vi "Plot menu activation.vi"(5 "panel mode":T1, 8 "error in (no error)":errorcluster, 9 "Coords":T5, 10 "Refs":T6, 11 "MenuRef":refnum<k9>) -> (0 "error out":errorcluster, 1 "Location":T2, 2 "Discard?":bool, 3 "MenuRef":refnum<k9>)   [LabVIEW 2021, in "RocketPlot.lvlib"]
uses:
  RocketPlot.lvlib
  Classes/RocketPlotHandle/RocketPlotHandle.lvclass
  TypeDefs/Plot UI references.ctl
  <userlib>/bjustice/TipStripOOPanel/Classes/TipPanelHandle/TipPanelHandle.lvclass
  TypeDefs/Plot top row.ctl
  <vilib>/Utility/miscctls.llb/LVPoint32TypeDef.ctl
  TypeDefs/Shortcut Location.ctl
  Plot menu activation submenu type v2.ctl
  TypeDefs/Plot axis.ctl
  Plot scale refnum to LUT name.vi
  TypeDefs/panel mode.ctl
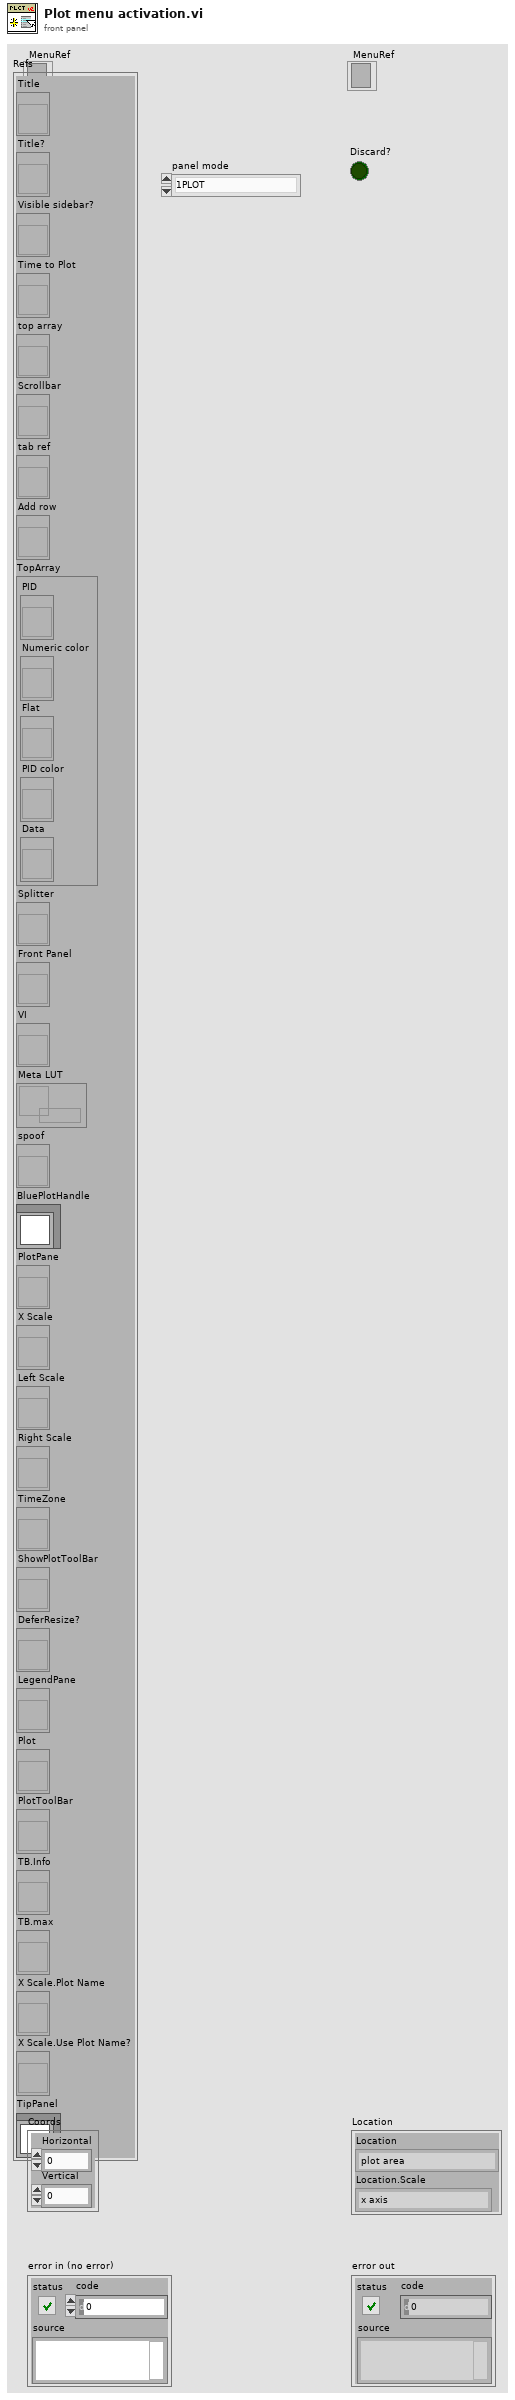
[diagram p1: front panel]
types:
  T1 = typedef "RocketPlot.lvlib/panel mode.ctl" = enum16{"1PLOT", "MPLOT"}
  T2 = typedef "RocketPlot.lvlib/Shortcut Location.ctl" = cluster{"Location":T3, "Location.Scale":T4}
  T3 = typedef "RocketPlot.lvlib/Plot menu activation submenu type v2.ctl" = enum16{"plot area", "plot border", "markers", "scale"}
  T4 = typedef "RocketPlot.lvlib/Plot axis.ctl" = enum16{"x axis", "left axis", "right axis"}
  T5 = typedef "LVPoint32TypeDef.ctl" = cluster{"Horizontal":i32, "Vertical":i32}
  T6 = typedef "RocketPlot.lvlib/Plot UI references.ctl" = cluster{"Title":refnum<vi>, "Title?":refnum<vi>, "Visible sidebar?":refnum<vi>, "Time to Plot":refnum<vi>, "top array":refnum<vi>, "Scrollbar":refnum<vi>, "tab ref":refnum<vi>, "Add row":refnum<vi>, "TopArray":cluster{"PID":refnum<vi>, "Numeric color":refnum<vi>, "Flat":refnum<vi>, "PID color":refnum<vi>, "Data":refnum<vi>}, "Splitter":refnum<vi>, "Front Panel":refnum<vi>, "VI":refnum<vi>, "Meta LUT":refnum<data-value>, "spoof":refnum<vi>, "BluePlotHandle":refnum<class "RocketPlotHandle.lvclass">, "PlotPane":refnum<vi>, "X Scale":refnum<vi>, "Left Scale":refnum<vi>, "Right Scale":refnum<vi>, "TimeZone":refnum<vi>, "ShowPlotToolBar":refnum<vi>, "DeferResize?":refnum<vi>, "LegendPane":refnum<vi>, "Plot":refnum<vi>, "PlotToolBar":refnum<vi>, "TB.Info":refnum<vi>, "TB.max":refnum<vi>, "X Scale.Plot Name":refnum<vi>, "X Scale.Use Plot Name?":refnum<vi>, "TipPanel":refnum<class "TipPanelHandle.lvclass">}
  T7 = typedef "RocketPlot.lvlib/PlatMods.ctl" = cluster{"Shift":bool, "Ctrl":bool, "Alt":bool}
  T8 = typedef "RocketPlot.lvlib/Plot scale meta JSON.ctl" = cluster{"Type":T4, "Grid Colors:Major Color":u32, "Grid Colors:Minor Color":u32, "Style":u8, "Tick Colors:Tick Color":u32, "Tick Colors:Minor Tick Color":u32, "Format String":string, "State":T9, "AxisFocus":refnum<vi>}
  T9 = typedef "RocketPlot.lvlib/Plot scale meta state.ctl" = cluster{"Visible":bool, "Focus":bool, "Multi-Y":bool}
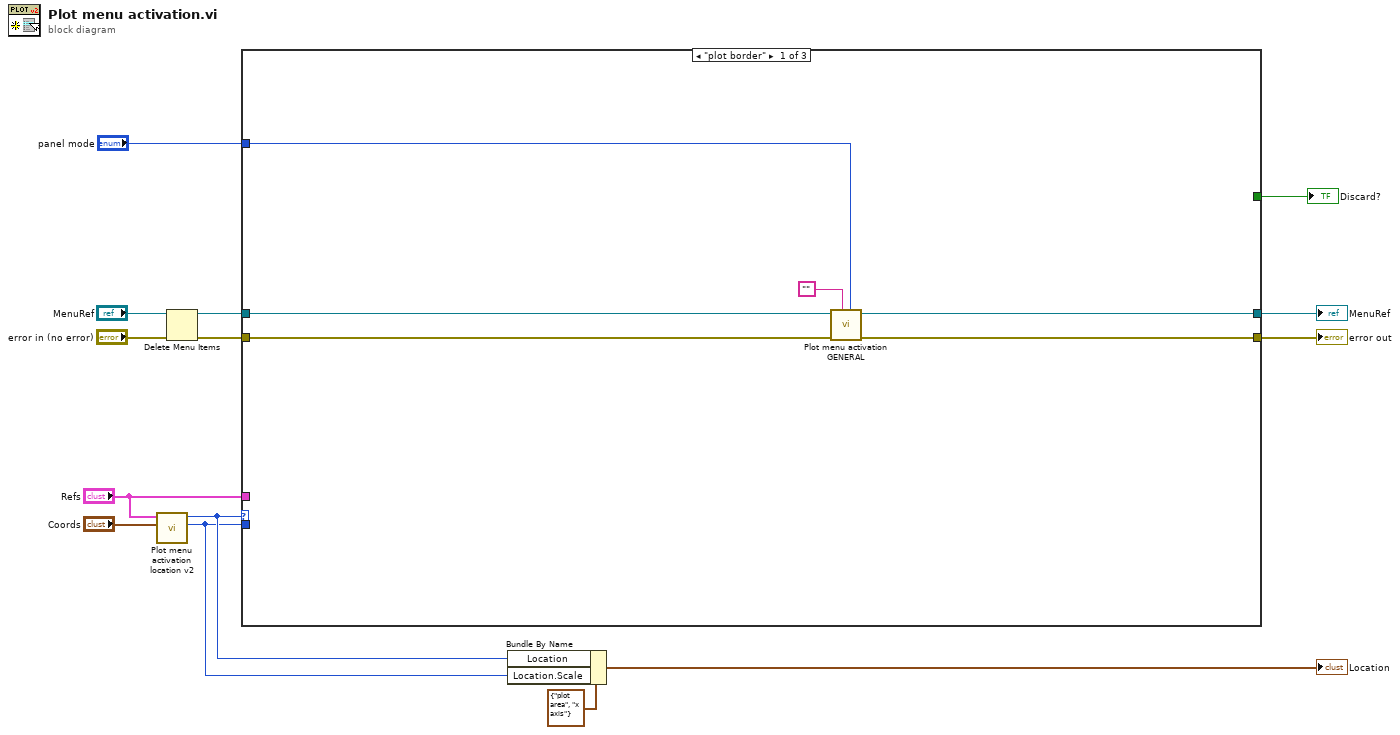
[diagram p0: block diagram]
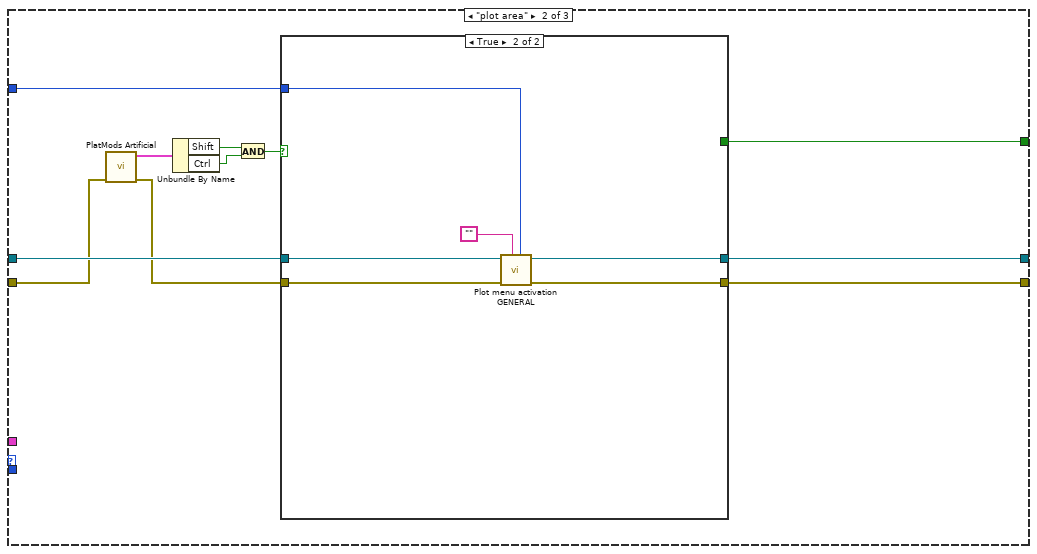
[diagram p2: hidden frame]
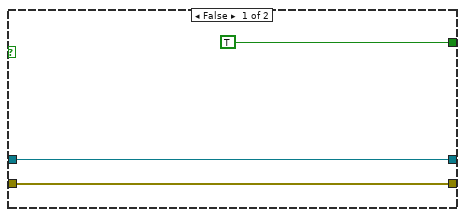
[diagram p3: hidden frame]
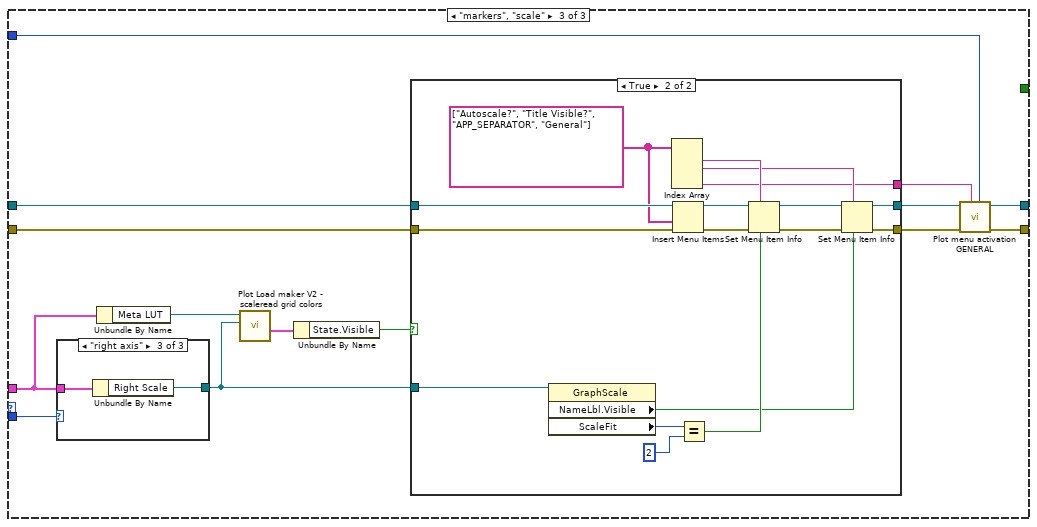
[diagram p4: hidden frame]
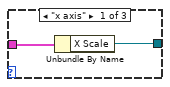
[diagram p6: hidden frame]
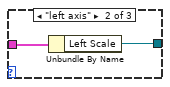
[diagram p7: hidden frame]
diagram:
  n1 = call "Plot menu activation location v2.vi"("Coords"="Coords", "Refs"="Refs") -> ("Location.Scale"=w4:T4, "Location"=w5:T3)  [unwired: 7 in, 1 out]
  n2 = Delete Menu Items(6:"error in (no error)", 9:"MenuRef") -> (0:w9:errorcluster, 3:w10:refnum<k9>)  [unwired: 2 in]
  n3 = case shown="\"plot border\"" w5 {
    tunnel: w4 -> [_ _ w54]
    tunnel: "Refs" -> [_ _ w46]
    tunnel: w10 -> [w18 w30 w53]
    tunnel: w9 -> [w20 w26 w52]
    tunnel: [w19 w31 w50] -> w8
    tunnel: [w16 w29 w47] -> w7
    tunnel: [_ w27 _] -> w2
    tunnel: "panel mode" -> [w15 w21 w41]
    frame "plot border" {
      n4 = call "Plot menu activation GENERAL.vi"("panel mode"=w15, "menu tag"="", "error in (no error)"=w20, "MenuRef"=w18) -> ("error out"=w19:errorcluster, "MenuRef"=w16:refnum<k9>)  [unwired: 6 in]
    }
    frame "plot area" {
      n5 = call "PlatMods Artificial.vi"("error in (no error)"=w26) -> ("error out"=w25:errorcluster, "PlatMods"=w28:T7)  [unwired: 9 in]
      n6 = Unbundle By Name(w28) -> ("Shift"=w24:bool, "Ctrl"=w23:bool)
      n7 = And(x=w24, y=w23) -> (x .and. y?=w22:bool)
      n8 = case shown="True" w22 {
        tunnel: w25 -> [w33 w40]
        tunnel: [w33 w39] -> w31
        tunnel: w30 -> [w34 w38]
        tunnel: [w34 w36] -> w29
        tunnel: [TRUE _] -> w27
        tunnel: w21 -> [_ w35]
        frame False {
        }
        frame True {
          n9 = call "Plot menu activation GENERAL.vi"("panel mode"=w35, "menu tag"="", "error in (no error)"=w40, "MenuRef"=w38) -> ("error out"=w39:errorcluster, "MenuRef"=w36:refnum<k9>)  [unwired: 6 in]
        }
      }
    }
    frame "markers", "scale" {
      n10 = case shown="\"right axis\"" w54 {
        tunnel: w46 -> [w75 w77 w79]
        tunnel: [w74 w76 w78] -> w44
        frame "x axis" {
          n11 = Unbundle By Name(w75) -> ("X Scale"=w74:refnum<vi>)
        }
        frame "left axis" {
          n12 = Unbundle By Name(w77) -> ("Left Scale"=w76:refnum<vi>)
        }
        frame "right axis" {
          n13 = Unbundle By Name(w79) -> ("Right Scale"=w78:refnum<vi>)
        }
      }
      n14 = Unbundle By Name(w46) -> ("Meta LUT"=w45:refnum<data-value>)
      n15 = call "Plot Load maker V2 - scaleread grid colors.vi"("Scale reference"=w44, "Meta LUT"=w45) -> ("Scale LUT meta"=w43:T8)  [unwired: 6 in, 3 out]
      n16 = Unbundle By Name(w43) -> ("State.Visible"=w42:bool)
      n17 = case shown="True" w42 {
        tunnel: w53 -> [w56 w73]
        tunnel: w52 -> [w55 w63]
        tunnel: [w55 w60] -> w51
        tunnel: [w56 w59] -> w49
        tunnel: [_ w58] -> w48
        tunnel: w44 -> [_ w57]
        frame False {
        }
        frame True {
          w71 = string[] ["Autoscale?", "Title Visible?", "APP_SEPARATOR", "General"]
          n18 = property class="GraphScale"(reference=w57) -> ("NameLbl.Visible"=w64:bool, "ScaleFit"=w69:u8)  [unwired: 1 in, 2 out]
          n19 = Index Array(array=w71) -> (element #1=w70:string, element #2=w65:string, element #4=w58:string)  [unwired: 4 in, 1 out]
          n20 = Insert Menu Items(6:w63, 7:w71, 9:w73) -> (0:w62:errorcluster, 3:w72:refnum<k9>)  [unwired: 3 in, 1 out]
          n21 = Equal?(x=w69, y=u8 2) -> (x = y?=w67:bool)
          n22 = Set Menu Item Info(6:w67, 7:w70, 8:w62, 11:w72) -> (0:w61:errorcluster, 3:w66:refnum<k9>)  [unwired: 3 in]
          n23 = Set Menu Item Info(6:w64, 7:w65, 8:w61, 11:w66) -> (0:w60:errorcluster, 3:w59:refnum<k9>)  [unwired: 3 in]
        }
      }
      n24 = call "Plot menu activation GENERAL.vi"("panel mode"=w41, "menu tag"=w48, "error in (no error)"=w51, "MenuRef"=w49) -> ("error out"=w50:errorcluster, "MenuRef"=w47:refnum<k9>)  [unwired: 6 in]
    }
  }
  "error out" <- w8
  "MenuRef" <- w7
  "Discard?" <- w2
  n25 = Bundle By Name(cluster=T2 {"Location"=enum."plot area", "Location.Scale"=enum."x axis"} ("Cluster"), "Location"=w5, "Location.Scale"=w4) -> (→"Location":T2)
